vi "digital read.vi"(8 "error in (no error)":errorcluster, 10 "Line":string, 11 "USB-6001 in":refnum<class "USB-6001.lvclass">) -> (0 "error out":errorcluster, 2 "High/Low":bool, 3 "USB-6001 out":refnum<class "USB-6001.lvclass">)   [LabVIEW 2025, in "USB IO.lvlib" / "USB-6001.lvclass"]
uses:
  USB-6001.lvclass
  USB-6001.lvclass/USB-6001.ctl
  <vilib>/DAQmx/read.llb/DAQmx Read (Digital Bool 1Line 1Point).vi
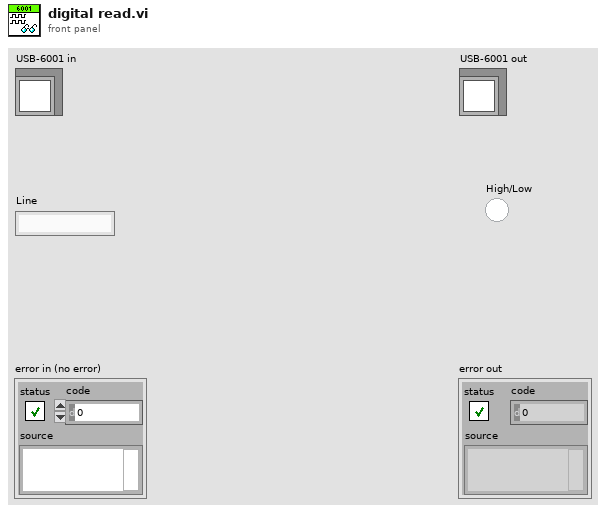
[diagram p1: front panel]
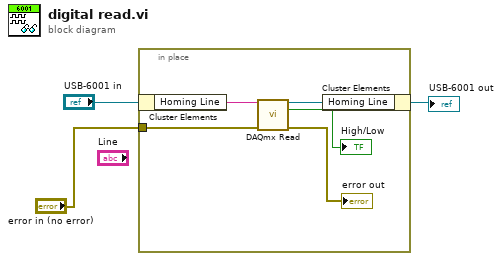
[diagram p0: block diagram]
diagram:
  n1 = in-place {
    in-place-border: "error in (no error)" -> [w6]
    n2 = in-place-cluster #1("USB-6001 in") -> ("Homing Line"=w8:string)
    n3 = call-poly <vilib>:"DAQmx Read.vi"("task/channels in"=w8, "error in"=w6) -> ("task out"=w7:refnum<k21>, "data"=→"High/Low":bool, "error out"=→"error out":errorcluster)  [unwired: 11 in]
    n4 = in-place-cluster #1("Homing Line"=w7) -> (→"USB-6001 out":refnum<class "USB-6001.lvclass">)
  }
